vi "Process.vi"(8 "error in":errorcluster, 11 "Qbus in":refnum<class "Qbus.lvclass">) -> (0 "error out":errorcluster)   [LabVIEW 2021, in "AudioGenManageConnectionProcess.lvlib"]
uses:
  AudioGenManageConnectionProcess.lvlib
  <vilib>/addons/Qbus/Qbus.lvclass
  shared/logger process/controls/event.ctl
  <vilib>/NI/STM/TCP/Write Meta Data (TCP Ref).vi
  <vilib>/NI/STM/TCP/Get Connection Reference (TCP).vi
  <vilib>/NI/STM/TCP/Write Meta Data (TCP Clst).vi
  <vilib>/NI/STM/TCP/Write Message (TCP).vi
  <vilib>/NI/STM/Connection Manager/TCP/TCP Connection Manager.vi
  shared/logger process/EventLoggerProcess.lvlib
  <vilib>/NI/STM/NI STM.lvlib
  subVIs/utility/AudioGenUtility.lvlib
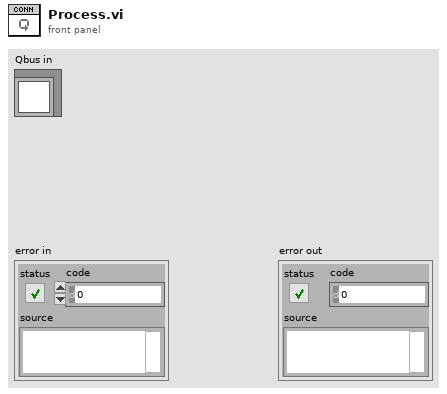
[diagram p1: front panel]
types:
  T1 = typedef "EventLoggerProcess.lvlib/event.ctl" = cluster{"name":string, "description":string}
  T2 = typedef "AudioGenTypeDefs.lvlib/service settings.ctl" = cluster{"port":u32, "enable debug log":bool}
  T3 = typedef "NI STM.lvlib/TCP Connection Info.ctl" = cluster{"connection ID":refnum<k5>, "meta data":T4[]}
  T4 = typedef "NI STM.lvlib/MetaDataElement.ctl" = string
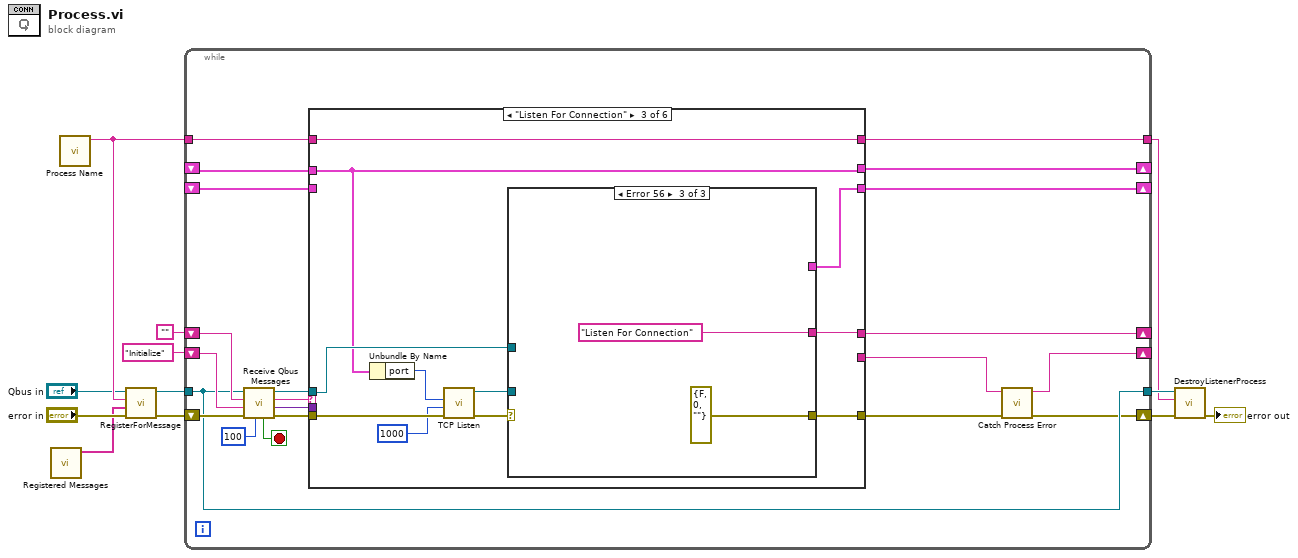
[diagram p0: block diagram]
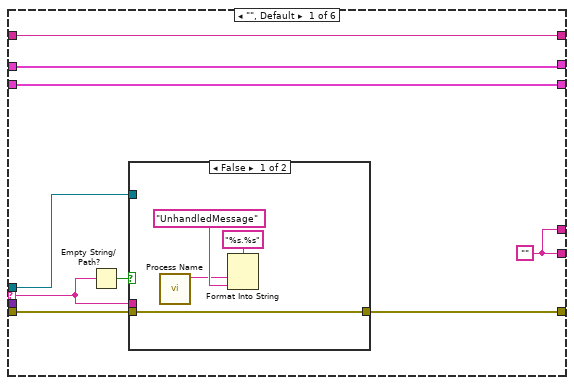
[diagram p2: hidden frame]
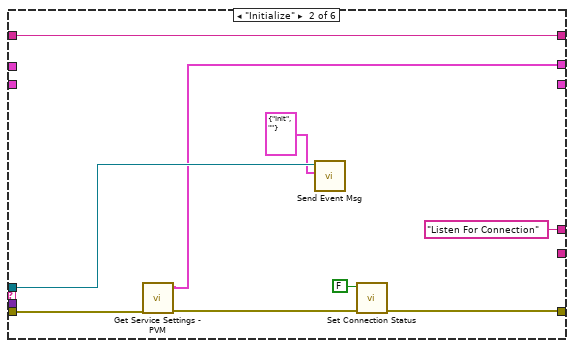
[diagram p4: hidden frame]
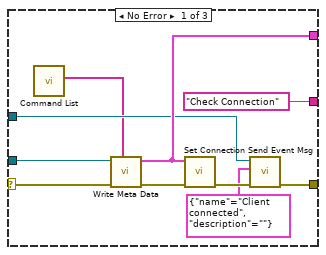
[diagram p5: hidden frame]
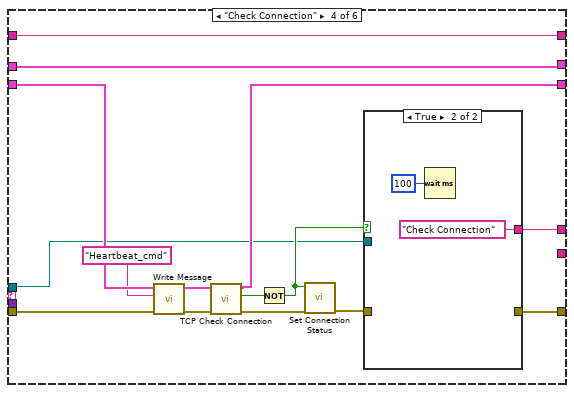
[diagram p7: hidden frame]
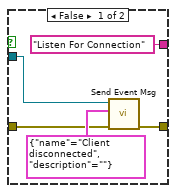
[diagram p8: hidden frame]
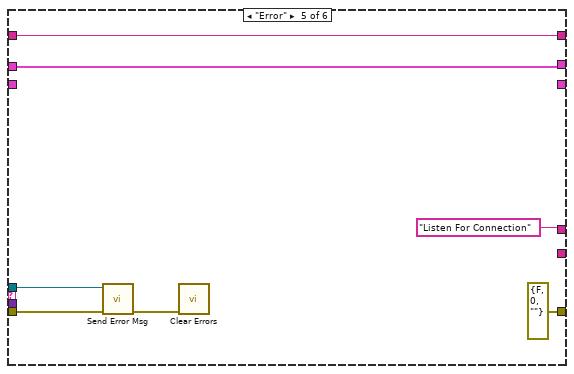
[diagram p9: hidden frame]
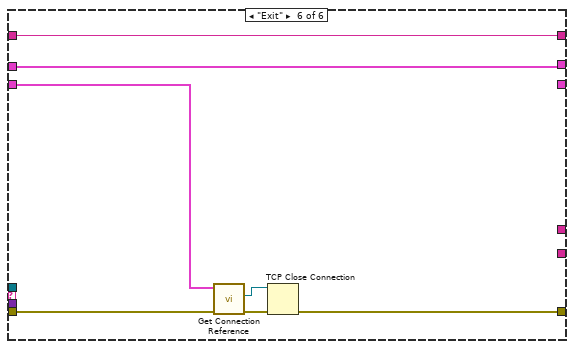
[diagram p10: hidden frame]
diagram:
  n1 = call "Registered Messages.vi"() -> ("registered messages"=w5:string[])  [unwired: 11 in]
  n2 = call "Process Name.vi"() -> ("process name"=w8:string)  [unwired: 11 in]
  n3 = call <vilib>:"RegisterForMessage.vi"("error in (no error)"="error in", "message names"=w5, "process name"=w8, "Qbus in"="Qbus in") -> ("error in (no error)"=w11:errorcluster, "Qbus out"=w12:refnum<class "Qbus.lvclass">)  [unwired: 6 in]
  n4 = while {
    shift-right: [w23] -> _
    shift-left: "" -> [w32]
    tunnel: w12 -> [w17]
    tunnel: w8 -> [w22]
    tunnel: [w17] -> w3
    tunnel: [w24] -> w1
    shift-right: [w14] -> _
    shift-left: "Initialize" -> [w28]
    shift-right: [w13] -> w4
    shift-left: w11 -> [w27]
    shift-right: [w21] -> _
    shift-left: _ -> [w20]
    shift-right: [w19] -> _
    shift-left: _ -> [w18]
    stop <- w33 stop-if-true
    n5 = call "Receive Qbus Messages.vi"("timeout(ms)"=100 ("milliseconds to wait"), "error in (no error)"=w27, "priority action"=w28, "default action"=w32, "Qbus in"=w17) -> ("error out"=w31:errorcluster, "message value"=w29:variant, "action"=w26:string, "Qbus out"=w30:refnum<class "Qbus.lvclass">, "exit"=w33:bool)  [unwired: 2 in]
    n6 = case shown="\"Listen For Connection\"" w26 {
      selector: w26 -> [w39 _ _ _ _ _]
      tunnel: w31 -> [w41 w50 w66 w94 w106 w113]
      tunnel: w30 -> [w37 w55 w59 w82 w105 _]
      tunnel: [w40 w52 w63 w89 errorcluster {"status"=FALSE, "code"=0, "source"=""} ("error out") w112] -> w16
      tunnel: w29 -> [_ _ _ _ _ _]
      tunnel: [w42 w56 w67 w95 w109 w116] -> w24
      tunnel: w22 -> [w42 w56 w67 w95 w109 w116]
      tunnel: [w36 _ _ _ _ _] -> w15
      tunnel: [w36 "Listen For Connection" w62 w88 "Listen For Connection" _] -> w23
      tunnel: [w35 _ w60 w87 _ _] -> w21
      tunnel: w20 -> [w35 _ _ w93 _ w111]
      tunnel: [w34 w48 w58 w81 w108 w110] -> w19
      tunnel: w18 -> [w34 _ w58 w81 w108 w110]
      frame "", Default {
        w36 = ""
        n7 = Empty String/Path?(string/path=w39) -> (empty?=w38:bool)
        n8 = case shown="False" w38 {
          tunnel: [w43 w47] -> w40
          tunnel: w41 -> [w43 w47]
          tunnel: w39 -> [_ _]
          tunnel: w37 -> [_ _]
          frame False {
            n9 = call "Process Name.vi"() -> ("process name"=w44:string)  [unwired: 11 in]
            n10 = Format Into String(format string="%s.%s", w44, "UnhandledMessage" ("ProcessName")) -> ()  [unwired: 2 in, 2 out]
          }
          frame True {
          }
        }
      }
      frame "Initialize" {
        n11 = call "Get Service Settings - PVM.vi"("error in (no error)"=w50) -> ("error out"=w49:errorcluster, "service settings"=w48:T2)  [unwired: 9 in]
        n12 = call "Send Event Msg.vi"("event"=T1 {"name"="Init", "description"=""}, "Qbus in"=w55) -> ()  [unwired: 8 in, 2 out]
        n13 = call "Set Connection Status.vi"("error in (no error)"=w49, "connected"=FALSE) -> ("error out"=w52:errorcluster)  [unwired: 9 in]
      }
      frame "Listen For Connection" {
        n14 = Unbundle By Name(w58) -> ("port"=w57:u32)
        n15 = call <vilib>:"TCP Listen.vi"("error in (no error)"=w66, "timeout ms (wait forever: -1)"=1000, "port"=w57) -> ("error out"=w64:errorcluster, "connection ID"=w61:refnum<k5>)  [unwired: 1 in, 6 out]
        n16 = case shown="Error 56" w64 {
          selector: w64 -> [w76 w78 _]
          tunnel: [w70 w78 errorcluster {"status"=FALSE, "code"=0, "source"=""} ("error IO")] -> w63
          tunnel: ["Check Connection" _ "Listen For Connection"] -> w62
          tunnel: w61 -> [w77 _ _]
          tunnel: [w73 _ _] -> w60
          tunnel: w59 -> [w71 _ _]
          frame No Error {
            n17 = call "Command List.vi"() -> ("TCP commands"=w68:string[])  [unwired: 11 in]
            n18 = call-poly <vilib>:"Write Meta Data.vi"("meta data"=w68, "error in"=w76, "connection ID"=w77) -> ("error out"=w74:errorcluster, "connection info out"=w73:T3)  [unwired: 2 in, 5 out]
            n19 = call "Set Connection.vi"("error in (no error)"=w74, "connection"=w73) -> ("error out"=w72:errorcluster)  [unwired: 9 in]
            n20 = call "Send Event Msg.vi"("error in"=w72, "event"=T1 {"name"="Client connected", "description"=""}, "Qbus in"=w71) -> ("error out"=w70:errorcluster)  [unwired: 7 in, 1 out]
          }
          frame Default {
          }
          frame Error {
          }
        }
      }
      frame "Check Connection" {
        n21 = call-poly <vilib>:"Write Message.vi"("error in"=w94, "name"="Heartbeat_cmd", "connection info in"=w93) -> ("error out"=w90:errorcluster, "connection info out"=w91:T3)  [unwired: 7 in]
        n22 = call <vilib>:"TCP Check Connection.vi"("error in"=w90, "connection in"=w91) -> ("error out"=w86:errorcluster, "disconnected?"=w84:bool, "connection out"=w87:T3)  [unwired: 7 in]
        n23 = Not(x=w84) -> (.not. x?=w83:bool)
        n24 = call "Set Connection Status.vi"("error in (no error)"=w86, "connected"=w83) -> ("error out"=w85:errorcluster)  [unwired: 9 in]
        n25 = case shown="True" w83 {
          tunnel: w85 -> [w98 _]
          tunnel: [w97 _] -> w89
          tunnel: ["Listen For Connection" "Check Connection"] -> w88
          tunnel: w82 -> [w96 _]
          frame False {
            n26 = call "Send Event Msg.vi"("error in"=w98, "event"=T1 {"name"="Client disconnected", "description"=""}, "Qbus in"=w96) -> ("error out"=w97:errorcluster)  [unwired: 7 in, 1 out]
          }
          frame True {
            n27 = Wait (ms)(milliseconds to wait=u32 100) -> ()  [unwired: 1 out]
          }
        }
      }
      frame "Error" {
        n28 = call "Send Error Msg.vi"("error in"=w106, "Qbus in"=w105) -> ("error out"=w104:errorcluster)  [unwired: 8 in, 1 out]
        n29 = call <vilib>:"Clear Errors.vi"("error in (no error)"=w104) -> ()  [unwired: 5 in, 2 out]
      }
      frame "Exit" {
        n30 = call-poly <vilib>:"Get Connection Reference.vi"("error in"=w113, "connection info in"=w111) -> ("error out"=w114:errorcluster, "connection ID out"=w115:refnum<k5>)  [unwired: 8 out]
        n31 = TCP Close Connection(connection ID=w115, error in (no error)=w114) -> (error out=w112:errorcluster)  [unwired: 2 out]
      }
    }
    n32 = call "Catch Process Error.vi"("error in (no error)"=w16, "priority action"=w15) -> ("error out"=w13:errorcluster, "priority action"=w14:string)  [unwired: 8 in]
  }
  n33 = call <vilib>:"DestroyListenerProcess.vi"("error in (no error)"=w4, "process name"=w1, "Qbus in"=w3) -> ("error in (no error)"=→"error out":errorcluster)  [unwired: 7 in, 1 out]
